vi "Conpane Probe A.vi"() -> ()   [LabVIEW 2026]
doc: "Round-13 connector-pane probe: y = x * factor. Identical in all four variants; only conIdx differs, so any difference in the connector pane is caused by conIdx and nothing else."
panel:
  out "y":dbl
  in  "factor":dbl=2.0
  in  "x":dbl=1.0
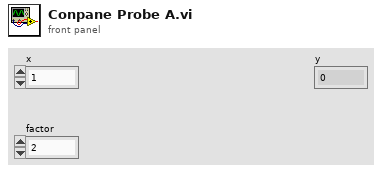
[diagram p1: front panel]
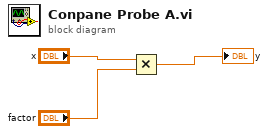
[diagram p0: block diagram]
diagram:
  n1 = Multiply(x="x", y="factor") -> (x*y=→"y":dbl)
